vi "LiftBin.vi"(0 "Position to Reach":dbl, 1 "NXT/EV3 IN":T1, 2 "Speed":dbl) -> (3 "NXT/EV3 OUT":T1)   [LabVIEW 2016, in "13.03 Robot.lvrbt"]
uses:
  13.03 Robot.lvrbt
  <vilib>/NXT/Subs/LVHSConnector.ctl
  <vilib>/NXT/LegoClasses/BrickReference/BrickReference.lvclass
  <vilib>/NXT/Block Support/NXT_OutputPort.ctl
  <vilib>/NXT/NXTIO Xnodes/NXTIONodeSubVIs/NXTMotorRunDistance.vi
  <vilib>/NXT/NXTIO Xnodes/AddressXNode/NXTIOAddress.xnode
  <vilib>/NXT/NXTIO Xnodes/NXTIOXNode/NXTIO.xnode
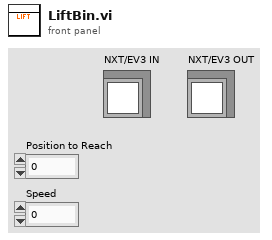
[diagram p1: front panel]
types:
  T1 = typedef "LVHSConnector.ctl" = refnum<class "BrickReference.lvclass">
  T2 = typedef "NXT_OutputPort.ctl" = u8
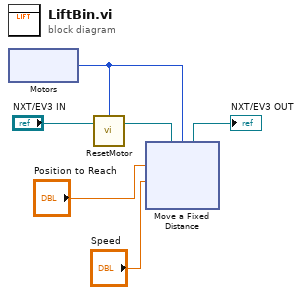
[diagram p0: block diagram]
diagram:
  n1 = xnode "Motors"() -> ("Motor"=w2:T2)
  n2 = call <vilib>:"ResetMotor.vi"("NXT/EV3"="NXT/EV3 IN", "Port (All Ports)"=w2) -> ("NXT/EV3"=w1:T1)  [unwired: 2 in]
  n3 = xnode "Move a Fixed Distance"("Speed 1"="Speed", "Distance 1"="Position to Reach", "Motors"=w2, "NXT/EV3"=w1) -> ("NXT/EV3"=→"NXT/EV3 OUT":T1)
